vi "ToDo.vi"   [LabVIEW 2014]
uses:
  MongoDB.Collection.lvclass
  C:/Users/Richard/Documents/GitHub/mongo-labview-driver/CSharp/bin/MongoDB.Driver.Legacy.dll
  CSharp/bin/MongoDB.Driver.Legacy.dll
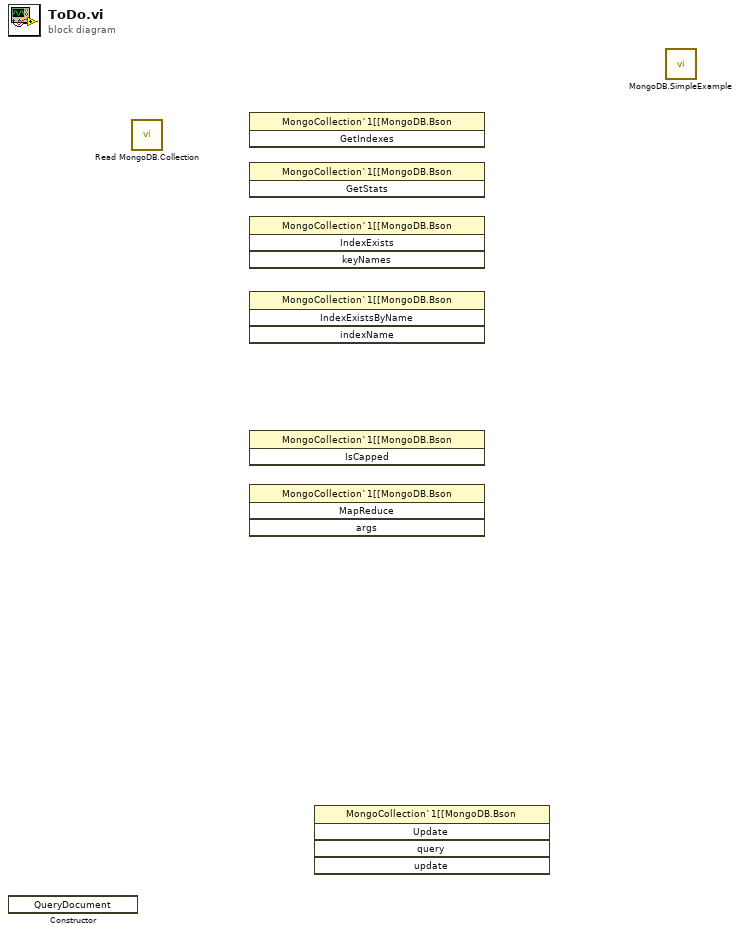
[diagram p0: block diagram]
diagram:
  n1 = constructor class="QueryDocument"() -> ()  [unwired: 3 in, 3 out]
  n2 = call "Read MongoDB.Collection.vi"() -> ()  [unwired: 9 in, 3 out]
  n3 = invoke class="MongoCollection`1[[MongoDB.Bson" method="GetIndexes"() -> ()  [unwired: 3 in, 3 out]
  n4 = invoke class="MongoCollection`1[[MongoDB.Bson" method="GetStats"() -> ()  [unwired: 3 in, 3 out]
  n5 = invoke class="MongoCollection`1[[MongoDB.Bson" method="IndexExists"() -> ()  [unwired: 4 in, 4 out]
  n6 = invoke class="MongoCollection`1[[MongoDB.Bson" method="IndexExistsByName"() -> ()  [unwired: 4 in, 4 out]
  n7 = invoke class="MongoCollection`1[[MongoDB.Bson" method="IsCapped"() -> ()  [unwired: 3 in, 3 out]
  n8 = invoke class="MongoCollection`1[[MongoDB.Bson" method="MapReduce"() -> ()  [unwired: 4 in, 4 out]
  n9 = invoke class="MongoCollection`1[[MongoDB.Bson" method="Update"() -> ()  [unwired: 5 in, 5 out]
  n10 = call "MongoDB.SimpleExample.vi"() -> ()  [unwired: 12 in]
